vi "VIH - CHM Project - Write Info File - Write.vi"(7 "Expect HHP exist (T)":bool=TRUE, 8 "error in":errorcluster, 9 "Project Files":T2, 10 "Files in HHP":T3, 11 "Target HHP File":path) -> (0 "error out":errorcluster, 2 "Info File":path)   [LabVIEW 2014]
doc: "::: VI Helpeks :::\nCopyright (c) 2000-2026 Konstantin Shifershteyn. All rights reserved."
uses:
  _VIH HelpGen - Palette.llb/VIH HelpGen Typedef - Palette - Item Type Enum.ctl
  <vilib>/Utility/config.llb/Write Key (String).vi
  <vilib>/Utility/config.llb/NI_LVConfig.lvlib
panel:
  # "VI Helpeks\nCopyright (c) 2012-2026 Konstantin Shifershteyn"
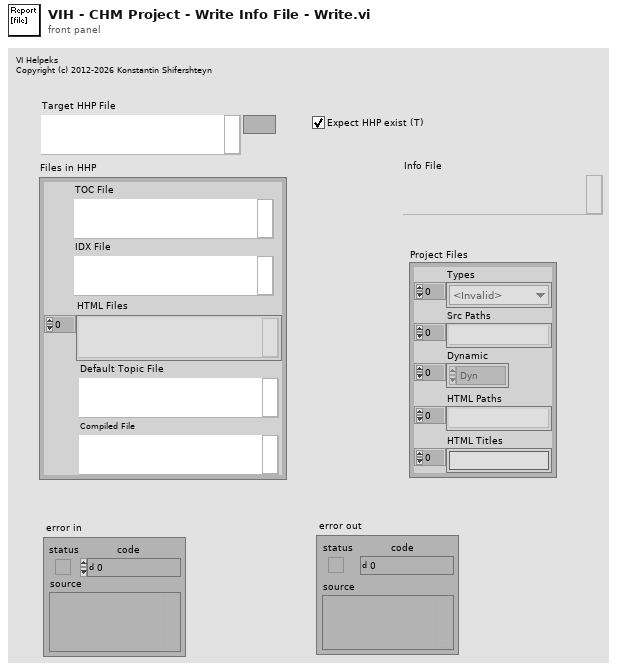
[diagram p1: front panel]
types:
  T1 = typedef "VIH HelpGen Typedef - Palette - Item Type Enum.ctl" = enum32{"<Invalid>", "<unknown>", "VI", "Menu", "LV Func", "Express VI", "Poly VI", "CTL", "HTML"}
  T2 = cluster{"Types":T1[], "Src Paths":path[], "Dynamic":enum16{"Dyn", "Stat", "Both"}[], "HTML Paths":path[], "HTML Titles":string[]}
  T3 = cluster{"TOC File":path, "IDX File":path, "HTML Files":path[], "Default Topic File":path, "Compiled File":path}
  T4 = typedef "NI_LVConfig.lvlib/Config Data RefNum.ctl" = refnum<k1>
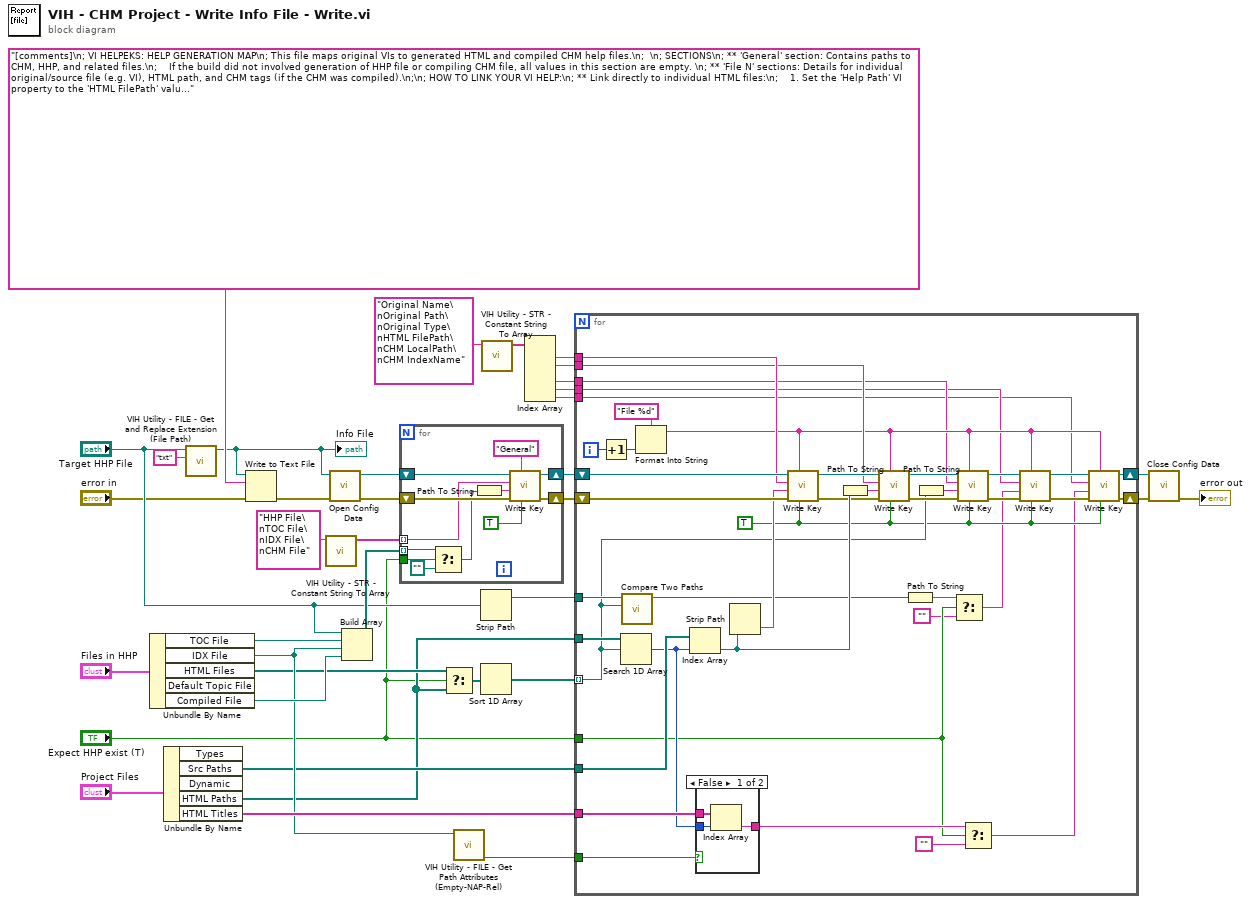
[diagram p0: block diagram]
diagram:
  n1 = Unbundle By Name("Files in HHP") -> ("TOC File"=w33:path, "IDX File"=w17:path, "HTML Files"=w5:path[], "Compiled File"=w32:path)  [unwired: 1 out]
  n2 = Unbundle By Name("Project Files") -> ("Src Paths"=w3:path[], "HTML Paths"=w2:path[], "HTML Titles"=w18:string[])  [unwired: 2 out]
  n3 = call "VIH Utility - FILE - Get and Replace Extension (File Path).vi"("new extension (none)"="txt", "file path"="Target HHP File") -> ("new file path"=w6:path)  [unwired: 8 in, 1 out]
  "Info File" <- w6
  n4 = Write to Text File(file (use dialog)=w6, text="[comments]\n; VI HELPEKS: HELP GENERATION MAP\n; This file maps original VIs to generated HTML and compiled CHM help files.\n;  \n; SECTIONS\n; ** 'General' section: Contains paths to CHM, HHP, and related files.\n;    If the build did not involved generation of HHP file or compiling CHM file, all values in this section are empty. \n; ** 'File N' sections: Details for individual original/source file (e.g. VI), HTML path, and CHM tags (if the CHM was compiled).\n;\n; HOW TO LINK YOUR VI HELP:\n; ** Link directly to individual HTML files:\n;    1. Set the 'Help Path' VI property to the 'HTML FilePath' value from a 'File N' section.\n;    2. Ensure the 'Help Tag' VI property is empty.\n; ** Link to compiled CHM file:\n;    1. Set the 'Help Path' VI property to the 'CHM File' value from the 'General' section.\n;    2. Set the 'Help Tag' VI property to either \"CHM LocalPath\" or \"CHM IndexName\" value from a 'File N' section.\n", error in="error in") -> (error out=w10:errorcluster)  [unwired: 1 in, 2 out]
  n5 = call "VIH Utility - STR - Constant String To Array.vi"("String in"="HHP File\nTOC File\nIDX File\nCHM File") -> ("Array out"=w35:string[])  [unwired: 10 in]
  n6 = call <vilib>:"Open Config Data.vi"("error in (no error)"=w10, "configuration file path"=w6) -> ("error out"=w7:errorcluster, "refnum"=w8:T4)  [unwired: 7 in, 1 out]
  n7 = Build Array("Target HHP File", w33, w17, w32) -> (w31:path[])
  n8 = for {
    shift-right: [w46] -> w30
    shift-left: w8 -> [w49]
    shift-right: [w45] -> w29
    shift-left: w7 -> [w48]
    tunnel: w35 -> [w44] mode=indexing
    tunnel: w31 -> [w41] mode=indexing
    tunnel: "Expect HHP exist (T)" -> [w38]
    n9 = Select(t=w41, s=w38, f=path "") -> (s? t:f=w40:path)
    n10 = Path To String(path=w40) -> (string=w43:string)
    n11 = call-poly <vilib>:"Write Key.vi"("write raw string? (F)"=TRUE, "section"="General", "error in (no error)"=w48, "value"=w43, "key"=w44, "refnum"=w49) -> ("error out"=w45:errorcluster, "refnum out"=w46:T4)  [unwired: 3 in, 1 out]
  }
  n12 = Select(t=w5, s="Expect HHP exist (T)", f=w2) -> (s? t:f=w4:path[])
  n13 = call "VIH Utility - FILE - Get Path Attributes (Empty-NAP-Rel).vi"("Path"=w17) -> ("Not A Path or Empty path"=w16:bool)  [unwired: 6 in, 4 out]
  n14 = Strip Path(path="Target HHP File") -> (stripped path=w21:path)  [unwired: 1 out]
  n15 = Sort 1D Array(array=w4) -> (sorted array=w12:path[])
  n16 = call "VIH Utility - STR - Constant String To Array.vi"("String in"="Original Name\nOriginal Path\nOriginal Type\nHTML FilePath\nCHM LocalPath\nCHM IndexName") -> ("Array out"=w26:string[])  [unwired: 10 in]
  n17 = Index Array(array=w26) -> (element #1=w25:string, element #2=w24:string, element #4=w23:string, element #5=w20:string, element #6=w19:string)  [unwired: 6 in, 1 out]
  n18 = for {
    tunnel: w12 -> [w68] mode=indexing
    tunnel: w2 -> [w85]
    tunnel: w3 -> [w84]
    tunnel: w25 -> [w83]
    tunnel: w24 -> [w80]
    tunnel: w23 -> [w70]
    tunnel: w21 -> [w69]
    tunnel: w20 -> [w66]
    tunnel: w19 -> [w65]
    tunnel: w18 -> [w64]
    shift-right: [w62] -> w15
    shift-left: w30 -> [w90]
    shift-right: [w61] -> w14
    shift-left: w29 -> [w89]
    tunnel: w16 -> [w60]
    tunnel: "Expect HHP exist (T)" -> [w52]
    i -> [w88]
    w57 = TRUE
    n19 = Increment(x=w88) -> (x+1=w87:i32)
    n20 = Search 1D Array(1D array=w85, element=w68) -> (index of element=w63:i32)  [unwired: 1 in]
    n21 = call <vilib>:"Compare Two Paths.vi"("Path 2"=w68, "Path 1"=w69) -> ("Relative Path from 1 to 2"=w67:path)  [unwired: 6 in, 3 out]
    n22 = Format Into String(format string="File %d", w87) -> (resulting string=w71:string)  [unwired: 2 in, 1 out]
    n23 = Index Array(array=w84, index=w63) -> (element=w79:path)
    n24 = case shown="False" w60 {
      tunnel: w64 -> [w93 _]
      tunnel: w63 -> [w92 _]
      tunnel: [w91 _] -> w54
      frame False {
        n25 = Index Array(array=w93, index=w92) -> (element=w91:string)
      }
      frame True {
      }
    }
    n26 = Strip Path(path=w79) -> (name=w82:string)  [unwired: 1 out]
    n27 = call-poly <vilib>:"Write Key.vi"("write raw string? (F)"=w57, "section"=w71, "error in (no error)"=w89, "value"=w82, "key"=w83, "refnum"=w90) -> ("error out"=w78:errorcluster, "refnum out"=w81:T4)  [unwired: 3 in, 1 out]
    n28 = Path To String(path=w79) -> (string=w59:string)
    n29 = call-poly <vilib>:"Write Key.vi"("write raw string? (F)"=w57, "section"=w71, "error in (no error)"=w78, "value"=w59, "key"=w80, "refnum"=w81) -> ("error out"=w74:errorcluster, "refnum out"=w77:T4)  [unwired: 3 in, 1 out]
    n30 = Path To String(path=w67) -> (string=w56:string)
    n31 = Path To String(path=w68) -> (string=w58:string)
    n32 = Select(t=w56, s=w52, f="") -> (s? t:f=w55:string)
    n33 = call-poly <vilib>:"Write Key.vi"("write raw string? (F)"=w57, "section"=w71, "error in (no error)"=w74, "value"=w58, "key"=w70, "refnum"=w77) -> ("error out"=w73:errorcluster, "refnum out"=w76:T4)  [unwired: 3 in, 1 out]
    n34 = Select(t=w54, s=w52, f="") -> (s? t:f=w53:string)
    n35 = call-poly <vilib>:"Write Key.vi"("write raw string? (F)"=w57, "section"=w71, "error in (no error)"=w73, "value"=w55, "key"=w66, "refnum"=w76) -> ("error out"=w72:errorcluster, "refnum out"=w75:T4)  [unwired: 3 in, 1 out]
    n36 = call-poly <vilib>:"Write Key.vi"("write raw string? (F)"=w57, "section"=w71, "error in (no error)"=w72, "value"=w53, "key"=w65, "refnum"=w75) -> ("error out"=w61:errorcluster, "refnum out"=w62:T4)  [unwired: 3 in, 1 out]
  }
  n37 = call <vilib>:"Close Config Data.vi"("error in (no error)"=w14, "refnum"=w15) -> ("error out"=→"error out":errorcluster)  [unwired: 8 in, 1 out]
